vi "Default Configuration.vi"() -> (3 "Default Configuration":T1={"Common"={"Period (s)"=0.2, "Offset (us)"=0, "Priority"=100, "Processor"=-2, "External Clock"={"ClockID"=0, "Clock Name"="", "Publish Clock"=FALSE, "Convert Data Timestamps"=FALSE, "Plugin Timing Source"=FALSE}}, "RX Interface"="CAN2", "Port Configuration"={"Mode"=enum."CAN FD", "Baud Rate"=500000, "Temination On"=TRUE, "Subordinate"=FALSE, "Echo TX"=FALSE, "FD Config"={"FD Baud Rate"=2000000, "ISO Mode"=TRUE, "BRS Enabled"=TRUE}}, "Timeout (ms)"=100, "Frames to read"=100, "Filter"={"Allow List (ID)"=[], "Deny List (ID)"=[]}} {"Filter"."Deny List (ID)" format="%.0x"; "Filter"."Allow List (ID)" format="%.0x"; "Port Configuration"."FD Config"."FD Baud Rate" format="%.0p"; "Port Configuration"."Baud Rate" format="%.0p"; "Common"."Period (s)" format="%#_13g"})   [LabVIEW 2021, in "CAN_Reader_NIXNET_Plugin.lvclass"]
uses:
  CAN_Reader_NIXNET_Plugin.lvclass
  Common/Typedef/Configuration.ctl
  <vilib>/CIF Foundation/CIF Core/CIFCore/Common/Typedef/Common Plugin Configuration.ctl
  <vilib>/CIF Foundation/CIF Core/CIFCore/Common/Typedef/External Clock Config.ctl
  <vilib>/CIF Foundation/CIF CAN RW Core/typedef/CAN Port Configuration.ctl
  <vilib>/CIF Foundation/CIF CAN RW Core/typedef/CAN Mode.ctl
  <vilib>/CIF Foundation/CIF CAN RW Core/typedef/FD Config.ctl
  <vilib>/CIF Foundation/CIF CAN RW Core/typedef/CAN Filter.ctl
  CAN_Reader_NIXNET_Plugin.lvclass/CAN_Reader_NIXNET_Plugin.ctl
  <vilib>/CIF Foundation/CIF Core/CIFCore/Common/CIFCoreCommon.lvlib
  Common/CAN_Reader_NIXNET_Common.lvlib
  <vilib>/CIF Foundation/CIF CAN RW Core/CAN_RW_CORE.lvclass
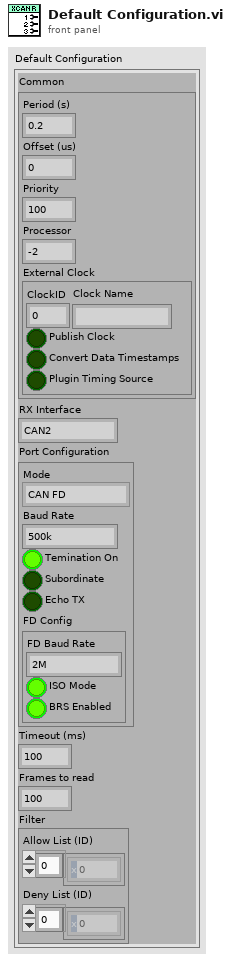
[diagram p1: front panel]
types:
  T1 = typedef "CAN_Reader_NIXNET_Common.lvlib/Configuration.ctl" = cluster{"Common":T2, "RX Interface":string, "Port Configuration":T4, "Timeout (ms)":i32, "Frames to read":i32, "Filter":T7}
  T2 = typedef "CIFCoreCommon.lvlib/Common Plugin Configuration.ctl" = cluster{"Period (s)":dbl, "Offset (us)":i32, "Priority":i32, "Processor":i32, "External Clock":T3}
  T3 = typedef "CIFCoreCommon.lvlib/External Clock Config.ctl" = cluster{"ClockID":u8, "Clock Name":string, "Publish Clock":bool, "Convert Data Timestamps":bool, "Plugin Timing Source":bool}
  T4 = typedef "CAN_RW_CORE.lvclass/CAN Port Configuration.ctl" = cluster{"Mode":T5, "Baud Rate":u64, "Temination On":bool, "Subordinate":bool, "Echo TX":bool, "FD Config":T6}
  T5 = typedef "CAN_RW_CORE.lvclass/CAN Mode.ctl" = enum16{"CAN 2.0", "CAN FD"}
  T6 = typedef "CAN_RW_CORE.lvclass/FD Config.ctl" = cluster{"FD Baud Rate":u64, "ISO Mode":bool, "BRS Enabled":bool}
  T7 = typedef "CAN_RW_CORE.lvclass/CAN Filter.ctl" = cluster{"Allow List (ID)":u32[], "Deny List (ID)":u32[]}
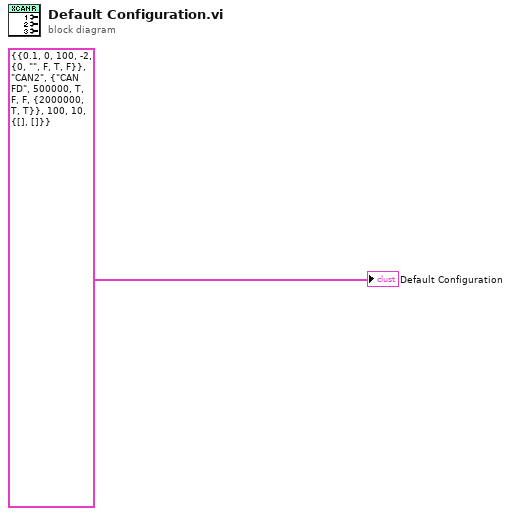
[diagram p0: block diagram]
diagram:
  "Default Configuration" <- T1 {"Common"={"Period (s)"=0.1, "Offset (us)"=0, "Priority"=100, "Processor"=-2, "External Clock"={"ClockID"=0, "Clock Name"="", "Publish Clock"=FALSE, "Convert Data Timestamps"=TRUE, "Plugin Timing Source"=FALSE}}, "RX Interface"="CAN2", "Port Configuration"={"Mode"=enum."CAN FD", "Baud Rate"=500000, "Temination On"=TRUE, "Subordinate"=FALSE, "Echo TX"=FALSE, "FD Config"={"FD Baud Rate"=2000000, "ISO Mode"=TRUE, "BRS Enabled"=TRUE}}, "Timeout (ms)"=100, "Frames to read"=10, "Filter"={"Allow List (ID)"=[], "Deny List (ID)"=[]}} ("Template Configuration")
